vi "Load User Devices.vi"(8 "error in (no error)":errorcluster, 11 "picoG in":refnum<class "picoG.lvclass">) -> (0 "error out":errorcluster, 3 "picoG out":refnum<class "picoG.lvclass">)   [LabVIEW 2020, in "PicoG-App.lvlib" / "picoG.lvclass"]
uses:
  picoG.lvclass
  picoG.lvclass/picoG.ctl
  DeviceListPanel/DeviceListPanel.lvclass
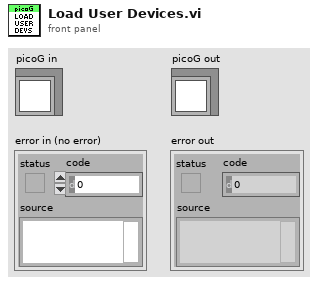
[diagram p1: front panel]
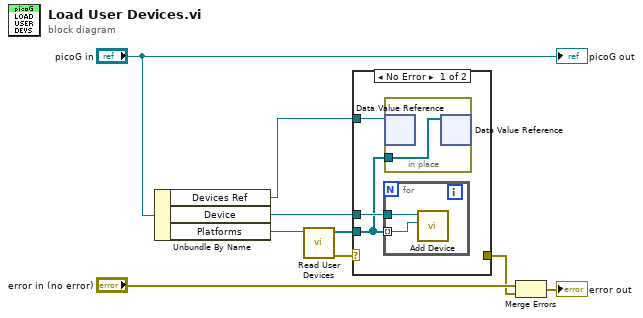
[diagram p0: block diagram]
diagram:
  n1 = Unbundle By Name("picoG in") -> ("Devices Ref"=w1:refnum<data-value>, "Device"=w6:refnum<class "DeviceListPanel.lvclass">, "Platforms"=w3:refnum<class "PlatformManager.lvclass">)
  n2 = call "Read User Devices.vi"("Platforms"=w3) -> ("error out"=w8:errorcluster, "User Devices"=w7:refnum<class "Device.lvclass">[])  [unwired: 9 in]
  n3 = case shown="No Error" w8 {
    selector: w8 -> [_ w16]
    tunnel: w7 -> [w10 _]
    tunnel: w6 -> [w12 _]
    tunnel: [_ w16] -> w4
    tunnel: w1 -> [w11 _]
    frame No Error {
      n4 = for {
        tunnel: w12 -> [w15]
        tunnel: w10 -> [w14] mode=indexing
        n5 = call "Add Device.vi"("Device"=w14, "DeviceListPanel in"=w15) -> ()  [unwired: 8 in, 2 out]
      }
      n6 = in-place {
        in-place-border: w10 -> [w13]
        n7 = in-place-dvr #1(w11) -> ()  [unwired: 2 out]
        n8 = in-place-dvr #1(w13) -> ()  [unwired: 2 out]
      }
    }
    frame Error {
    }
  }
  n9 = Merge Errors("error in (no error)", w4) -> (→"error out":errorcluster)
  "picoG out" <- "picoG in"
